vi "get_sine_point_from_array__f00654564c.vi"(8 "Initial position in voltage":dbl, 9 "voltage to displacement constant":dbl, 10 "sinewave point":dbl) -> (1 "String":string, 3 "Numeric":dbl)   [LabVIEW 2023]
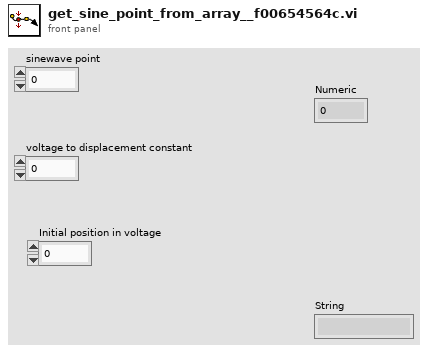
[diagram p1: front panel]
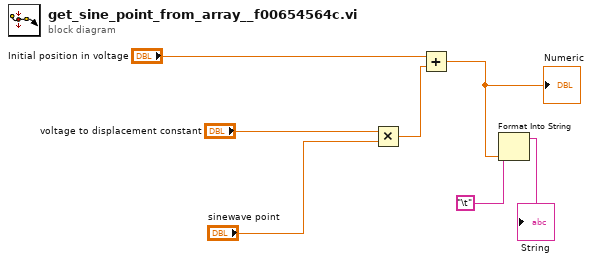
[diagram p0: block diagram]
diagram:
  n1 = Multiply(x="voltage to displacement constant", y="sinewave point") -> (x*y=w2:dbl)
  n2 = Add(x="Initial position in voltage", y=w2) -> (x+y=w7:dbl)
  "Numeric" <- w7
  n3 = Format Into String(initial string="\t", w7) -> (resulting string=→"String":string)  [unwired: 2 in, 1 out]
